vi "SA set Trace Det.vi"(8 "error in (no error)":errorcluster caption="에러 입력(에러 없음)", 10 "Detector Type":T1, 11 "Instrument Manager 입력":refnum<class "Instrument Manager.lvclass">) -> (0 "error out":errorcluster caption="에러 출력", 3 "Instrument Manager 출력":refnum<class "Instrument Manager.lvclass">)   [LabVIEW 2023, in "Instrument Manager.lvclass"]
uses:
  Instrument Manager.lvclass
  Instrument Manager.lvclass/Instrument Manager.ctl
  Module/Spectrum Analyzer/Interface_Spectrum/Interface_Spectrum.lvclass
  Module/Spectrum Analyzer/TYPE DEFINITION/TYPE Detect Mode Select.ctl
  Module/Spectrum Analyzer/Spectrum Analyzer.lvlib
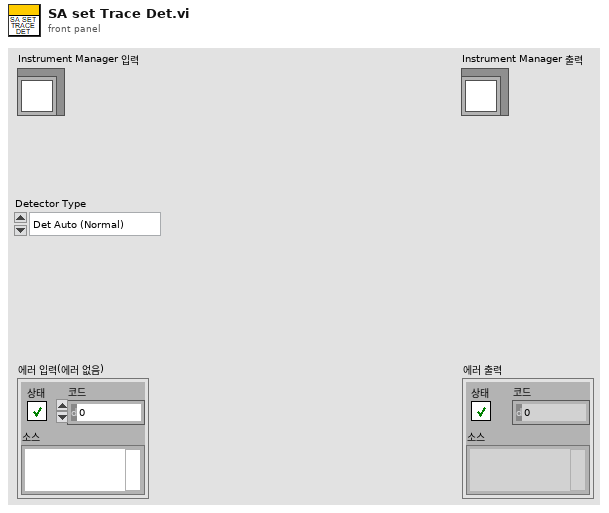
[diagram p1: front panel]
types:
  T1 = typedef "Spectrum Analyzer.lvlib/TYPE Detect Mode Select.ctl" = enum16{"Det Auto (Normal)", "Auto Peak", "Positive Peak", "Negative Peak", "Sample", "RMS", "Average", "Quasipeak", "CISPR Average", "RMS Average"}
  T2 = cluster{"Anritsu Call Box":refnum<class "Anritsu Call Box.lvclass">, "Spectrum Analyzer":refnum<class "Interface_Spectrum.lvclass">, "RF Switch Box":refnum<class "RF Filter Box.lvclass">, "Turn Table":refnum<class "Interface - Turn Table.lvclass">, "Mast":refnum<class "Interface - Mast.lvclass">, "3D Controller":refnum<class "Interface_3D Controller.lvclass">}
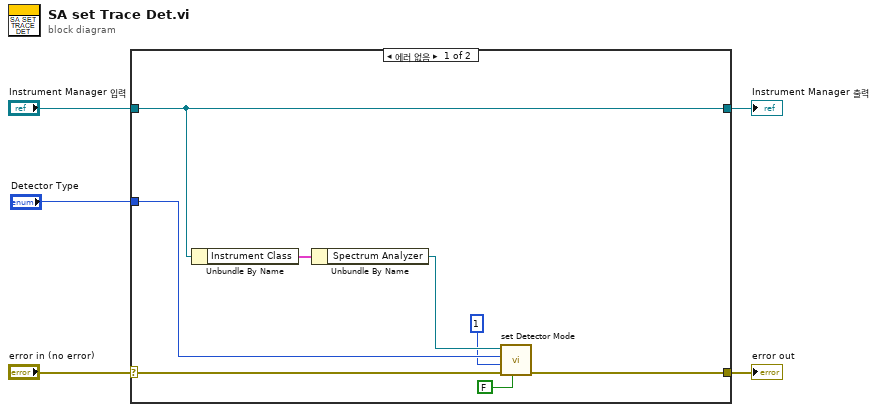
[diagram p0: block diagram]
diagram:
  n1 = case shown="에러 없음" "error in (no error)" {
    selector: "error in (no error)" -> [w11 w15]
    tunnel: [w10 w15] -> w4
    tunnel: [w13 w14] -> w2
    tunnel: "Instrument Manager 입력" -> [w13 w14]
    tunnel: "Detector Type" -> [w8 _]
    frame No Error {
      n2 = Unbundle By Name(w13) -> ("Instrument Class"=w12:T2)
      n3 = Unbundle By Name(w12) -> ("Spectrum Analyzer"=w9:refnum<class "Interface_Spectrum.lvclass">)
      n4 = call-dynamic "set Detector Mode.vi"("Detect Auto?"=FALSE, "error in (no error)"=w11, "Trace Index"=u32 1, "Detector Type"=w8, "Interface_Spectrum in"=w9) -> ("error out"=w10:errorcluster)  [unwired: 5 in, 1 out]
    }
    frame Error {
    }
  }
  "error out" <- w4
  "Instrument Manager 출력" <- w2
